vi "change CLFN properties.vi"() -> ()   [LabVIEW 2019]
uses:
  <vilib>/Utility/traverseref.llb/TRef TravTarget.ctl
  ca4436d5-b66f-4770-9057-43c195b94ee2.vi
  <vilib>/Utility/traverseref.llb/VI Scripting - Traverse.lvlib
panel:
  in  "Item(s) to Update":i32[](listbox)
  in  "PGconn/PGresults Type":enum16{"U32", "U64", "Pointer-Size"}(ring)
  out "Functions used":string[](array[string])
  in  "ShowMod":bool=TRUE caption="Open modified diagrams"
  in  "ApplyMod":bool=TRUE caption="Apply modifications"
  in  "Dynamic  Library":bool=TRUE
  in  "Call convention":enum16{"C", "stdcall"}(ring)
  in  "LibPath":string="libpq.*"
  out "Mod":path[](array[path]) caption="Modified VIs"
  in  "AnyThread":bool
  in  "folder":path=path "C:/dev/pq-labview"
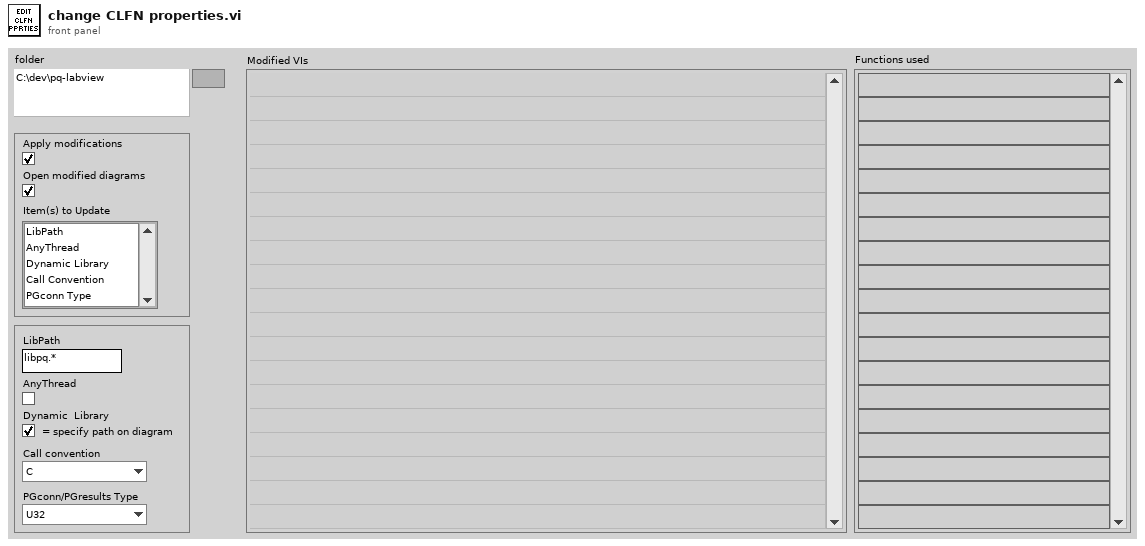
[diagram p1: front panel]
types:
  T1 = cluster{"AnyThread":bool, "LibPath":path, "Call Convention":u32, "Dynamic Library":bool, "PGconn Type":enum16{"I8", "I16", "I32", "I64", "U8", "U16", "U32", "U64", "SGL", "DBL", "PTR INT", "PTR UINT"}}
  T2 = enum16{"I8", "I16", "I32", "I64", "U8", "U16", "U32", "U64", "SGL", "DBL", "PTR INT", "PTR UINT"}
  T3 = typedef "TRef TravTarget.ctl" = enum16{"FP", "BD", "Other"}
  T4 = cluster{"Parameter Name":string, "Num Dimensions":i32, "Parameter Type":enum16{"Numeric", "Array", "String", "Waveform", "Digital Waveform", "Digital Table", "ActiveX", "Any", "Instance Data Pointer", "Void"}, "Numeric Type":enum16{"I8", "I16", "I32", "I64", "U8", "U16", "U32", "U64", "SGL", "DBL", "PTR INT", "PTR UINT"}, "Param Passing":enum16{"By Value", "Pointer To Value"}, "Array Passing":enum16{"Array Data Pointer", "Array Handle", "Array Handle Pointer"}, "String Passing":enum16{"C String Pointer", "Pascal String Pointer", "String Handle", "String Handle Pointer"}, "Adapt Format":enum16{"By Value", "Pointer To Value"}, "ActiveX Types":enum16{"ActiveX Variant Pointer", "IDispatch* Pointer", "IUnknown* Pointer"}, "Const (unused)":bool, "Minimum Size":string}[]
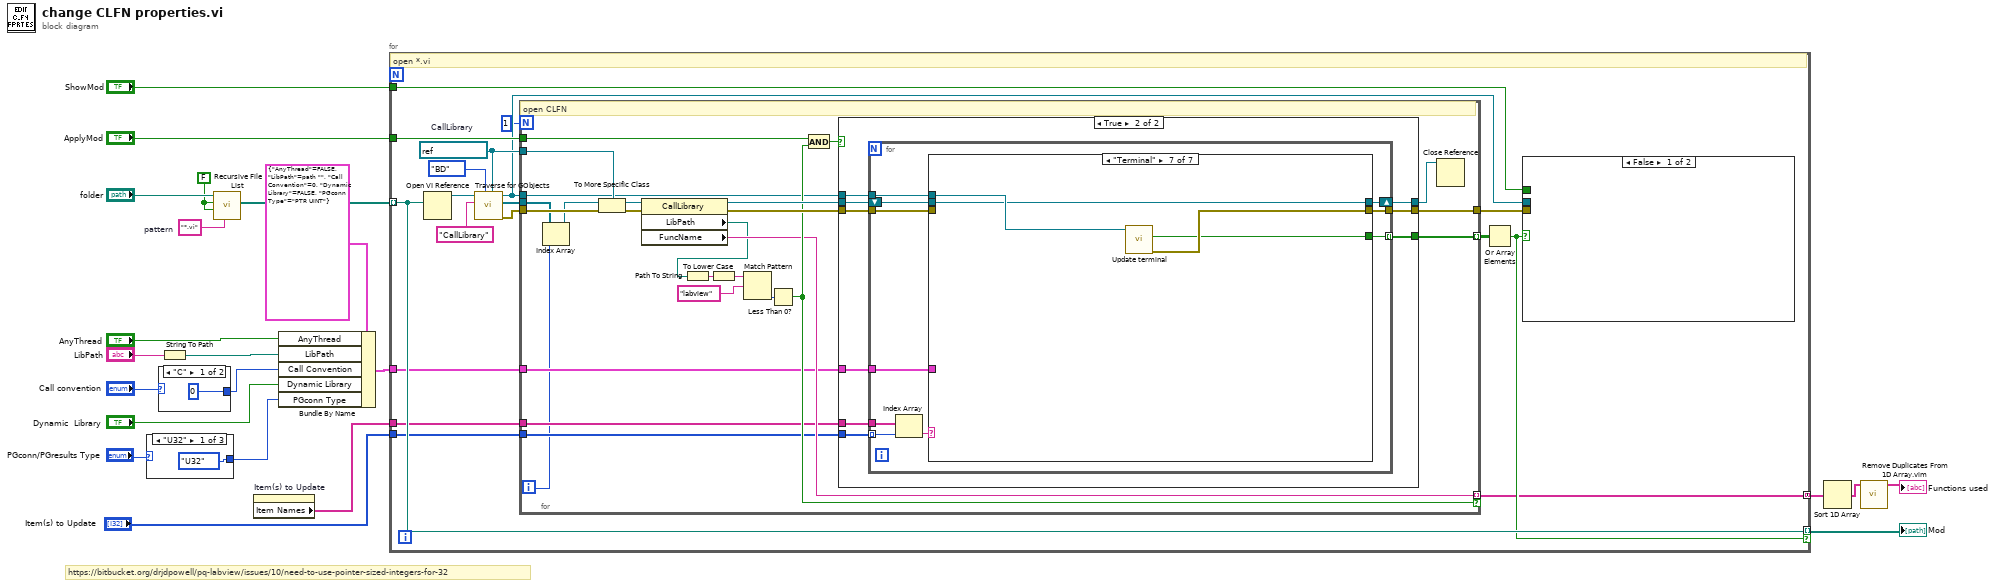
[diagram p0: block diagram]
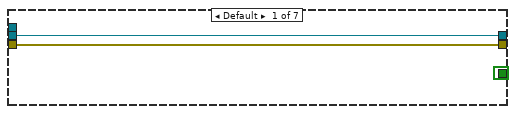
[diagram p3: hidden frame]
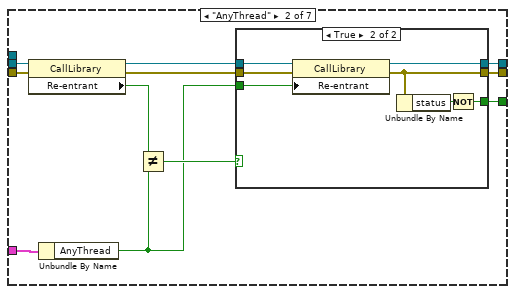
[diagram p4: hidden frame]
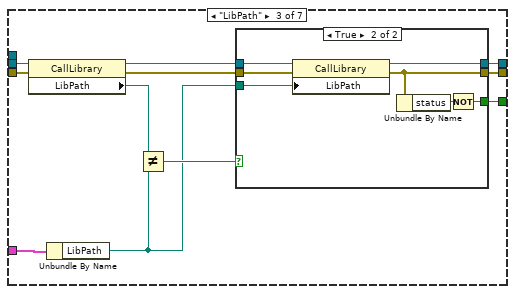
[diagram p6: hidden frame]
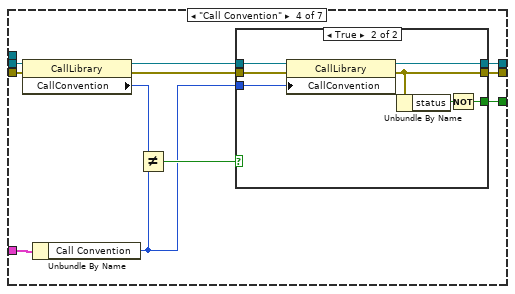
[diagram p8: hidden frame]
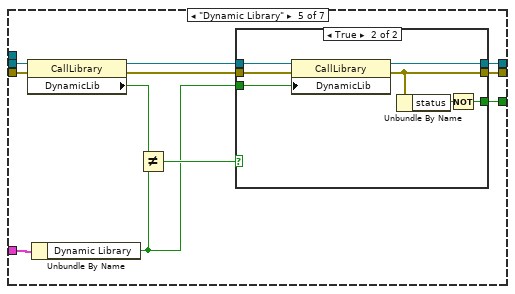
[diagram p10: hidden frame]
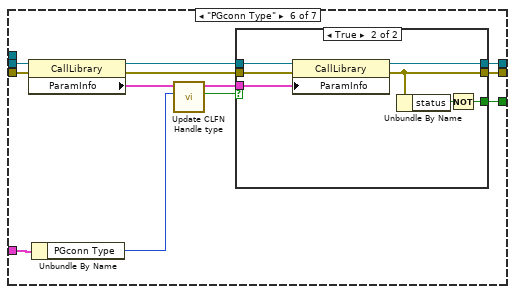
[diagram p12: hidden frame]
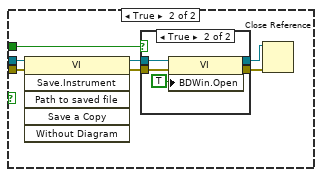
[diagram p14: hidden frame]
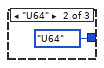
[diagram p16: hidden frame]
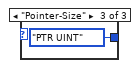
[diagram p17: hidden frame]
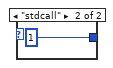
[diagram p18: hidden frame]
diagram:
  w20 = FALSE
  w19 = "*.vi"  # pattern
  # "https://bitbucket.org/drjdpowell/pq-labview/issues/10/need-to-use-pointer-sized-integers-for-32"
  n1 = case shown="\"U32\"" "PGconn/PGresults Type" {
    tunnel: [T2."U32" ("Numeric Type") T2."U64" ("Numeric Type") T2."PTR UINT" ("Numeric Type")] -> w4
    frame "U32" {
    }
    frame "U64" {
    }
    frame "Pointer-Size" {
    }
  }
  n2 = case shown="\"C\"" "Call convention" {
    tunnel: [u32 0 ("Calling Convention") u32 1 ("Calling Convention")] -> w6
    frame "C" {
    }
    frame "stdcall" {
    }
  }
  n3 = String To Path(string="LibPath") -> (path=w7:path)
  n4 = call <vilib>:"Recursive File List.vi"("pattern"=w19, "Continue Recursing on Error? (F)"=w20, "Treat LLBs as Folders?"=w20, "Folder Path"="folder") -> ("All Files in Dir"=w18:path[])  [unwired: 3 in, 4 out]
  n5 = property on="Item(s) to Update" class="LstBox (strict)"() -> ("Item Names"=w1:string[])  [unwired: 2 in, 2 out]
  n6 = Bundle By Name(cluster=T1 {"AnyThread"=FALSE, "LibPath"=path "", "Call Convention"=0, "Dynamic Library"=FALSE, "PGconn Type"=enum."PTR UINT"} ("output cluster"), "AnyThread"="AnyThread", "LibPath"=w7, "Call Convention"=w6, "Dynamic Library"="Dynamic  Library", "PGconn Type"=w4) -> (w5:T1)
  n7 = for {
    tunnel: w18 -> [w38] mode=indexing
    tunnel: [w38] -> w22 mode=indexing if=w34
    tunnel: "ApplyMod" -> [w37]
    tunnel: "ShowMod" -> [w36]
    tunnel: [w33] -> w13 mode=concatenating
    tunnel: w5 -> [w32]
    tunnel: "Item(s) to Update" -> [w31]
    tunnel: w1 -> [w30]
    w42 = refnum<vi> refnum  # CallLibrary
    # "open *.vi"
    n8 = Open VI Reference(vi path=w38) -> (vi reference=w45:refnum<vi>)  [unwired: 5 in, 1 out]
    n9 = call <vilib>:"Traverse for GObjects.vi"("Other Refnum"=w42, "Traverse Target"=TRef_TravTarget."BD", "Class Name"="CallLibrary", "VI Refnum"=w45) -> ("error out"=w41:errorcluster, "References"=w39:refnum<vi>[], "dup VI Refnum"=w29:refnum<vi>)  [unwired: 4 in, 1 out]
    n10 = for {
      N: 1 -> [_]
      tunnel: w39 -> [w46]
      tunnel: w42 -> [w70]
      tunnel: w41 -> [w69]
      tunnel: [w68] -> w40
      tunnel: w37 -> [w66]
      tunnel: [w65] -> w35 mode=indexing
      tunnel: [w54] -> w33 mode=indexing if=w55
      tunnel: w32 -> [w52]
      tunnel: w31 -> [w51]
      tunnel: w30 -> [w50]
      tunnel: w29 -> [w49]
      i -> [w48]
      # "open CLFN"
      n11 = Index Array(array=w46, index=w48) -> (element=w47:refnum<vi>)
      n12 = To More Specific Class(target class=w70, reference=w47, error in=w69) -> (specific class reference=w64:refnum<vi>, error out=w63:errorcluster)
      n13 = property class="CallLibrary"(reference=w64, error in=w63) -> (reference out=w62:refnum<vi>, error out=w61:errorcluster, "LibPath"=w53:path, "FuncName"=w54:string)
      n14 = Path To String(path=w53) -> (string=w60:string)
      n15 = To Lower Case(string=w60) -> (all lower case string=w59:string)
      n16 = Match Pattern(string=w59, regular expression="labview") -> (offset past match=w57:i32)  [unwired: 1 in, 3 out]
      n17 = Less Than 0?(x=w57) -> (x < 0?=w55:bool)
      n18 = Compound Arithmetic op=AND(w66, w55) -> (w56:bool)
      n19 = case shown="True" w56 {
        tunnel: w62 -> [w72 w79]
        tunnel: w61 -> [w71 w78]
        tunnel: [w71 w81] -> w68
        tunnel: [w72 w80] -> w67
        tunnel: [_ w77] -> w65
        tunnel: w52 -> [_ w76]
        tunnel: w51 -> [_ w75]
        tunnel: w50 -> [_ w74]
        tunnel: w49 -> [_ w73]
        frame False {
        }
        frame True {
          n20 = for {
            shift-right: [w90] -> w80
            shift-left: w79 -> [w89]
            tunnel: w78 -> [w88]
            tunnel: [w91] -> w81
            tunnel: [w87] -> w77 mode=indexing
            tunnel: w76 -> [w83]
            tunnel: w75 -> [w85] mode=indexing
            tunnel: w74 -> [w86]
            tunnel: w73 -> [w82]
            n21 = Index Array(array=w86, index=w85) -> (element=w84:string)
            n22 = case shown="\"Terminal\"" w84 {
              tunnel: [w93 w105 w125 w145 w165 w186 w198] -> w91
              tunnel: [w94 w104 w124 w144 w164 w185 w197] -> w90
              tunnel: w89 -> [w94 w103 w123 w143 w163 w184 w197]
              tunnel: w88 -> [w93 w100 w120 w140 w160 w181 _]
              tunnel: [FALSE w99 w119 w139 w159 w180 w196] -> w87
              tunnel: w83 -> [_ w98 w117 w137 w157 w177 _]
              tunnel: w82 -> [_ _ _ _ _ _ w199]
              frame Default {
              }
              frame "AnyThread" {
                n23 = property class="CallLibrary"(reference=w103, error in=w100) -> (reference out=w102:refnum<vi>, error out=w101:errorcluster, "Re-entrant"=w97:bool)
                n24 = Unbundle By Name(w98) -> ("AnyThread"=w95:bool)
                n25 = Not Equal?(x=w97, y=w95) -> (x != y?=w96:bool)
                n26 = case shown="True" w96 {
                  tunnel: [w106 w111] -> w105
                  tunnel: [w107 w114] -> w104
                  tunnel: w102 -> [w107 w113]
                  tunnel: w101 -> [w106 w112]
                  tunnel: [_ w109] -> w99
                  tunnel: w95 -> [_ w108]
                  frame False {
                  }
                  frame True {
                    n27 = property class="CallLibrary"(reference=w113, error in=w112, "Re-entrant"=w108) -> (reference out=w114:refnum<vi>, error out=w111:errorcluster)
                    n28 = Unbundle By Name(w111) -> ("status"=w110:bool)
                    n29 = Not(x=w110) -> (.not. x?=w109:bool)
                  }
                }
              }
              frame "LibPath" {
                n30 = property class="CallLibrary"(reference=w123, error in=w120) -> (reference out=w122:refnum<vi>, error out=w121:errorcluster, "LibPath"=w116:path)
                n31 = Unbundle By Name(w117) -> ("LibPath"=w115:path)
                n32 = Not Equal?(x=w116, y=w115) -> (x != y?=w118:bool)
                n33 = case shown="True" w118 {
                  tunnel: [w126 w131] -> w125
                  tunnel: [w127 w134] -> w124
                  tunnel: w122 -> [w127 w133]
                  tunnel: w121 -> [w126 w132]
                  tunnel: [_ w129] -> w119
                  tunnel: w115 -> [_ w128]
                  frame False {
                  }
                  frame True {
                    n34 = property class="CallLibrary"(reference=w133, error in=w132, "LibPath"=w128) -> (reference out=w134:refnum<vi>, error out=w131:errorcluster)
                    n35 = Unbundle By Name(w131) -> ("status"=w130:bool)
                    n36 = Not(x=w130) -> (.not. x?=w129:bool)
                  }
                }
              }
              frame "Call Convention" {
                n37 = property class="CallLibrary"(reference=w143, error in=w140) -> (reference out=w142:refnum<vi>, error out=w141:errorcluster, "CallConvention"=w136:u32)
                n38 = Unbundle By Name(w137) -> ("Call Convention"=w135:u32)
                n39 = Not Equal?(x=w136, y=w135) -> (x != y?=w138:bool)
                n40 = case shown="True" w138 {
                  tunnel: [w146 w151] -> w145
                  tunnel: [w147 w154] -> w144
                  tunnel: w142 -> [w147 w153]
                  tunnel: w141 -> [w146 w152]
                  tunnel: [_ w149] -> w139
                  tunnel: w135 -> [_ w148]
                  frame False {
                  }
                  frame True {
                    n41 = property class="CallLibrary"(reference=w153, error in=w152, "CallConvention"=w148) -> (reference out=w154:refnum<vi>, error out=w151:errorcluster)
                    n42 = Unbundle By Name(w151) -> ("status"=w150:bool)
                    n43 = Not(x=w150) -> (.not. x?=w149:bool)
                  }
                }
              }
              frame "Dynamic Library" {
                n44 = property class="CallLibrary"(reference=w163, error in=w160) -> (reference out=w162:refnum<vi>, error out=w161:errorcluster, "DynamicLib"=w156:bool)
                n45 = Unbundle By Name(w157) -> ("Dynamic Library"=w155:bool)
                n46 = Not Equal?(x=w156, y=w155) -> (x != y?=w158:bool)
                n47 = case shown="True" w158 {
                  tunnel: [w166 w171] -> w165
                  tunnel: [w167 w174] -> w164
                  tunnel: w162 -> [w167 w173]
                  tunnel: w161 -> [w166 w172]
                  tunnel: [_ w169] -> w159
                  tunnel: w155 -> [_ w168]
                  frame False {
                  }
                  frame True {
                    n48 = property class="CallLibrary"(reference=w173, error in=w172, "DynamicLib"=w168) -> (reference out=w174:refnum<vi>, error out=w171:errorcluster)
                    n49 = Unbundle By Name(w171) -> ("status"=w170:bool)
                    n50 = Not(x=w170) -> (.not. x?=w169:bool)
                  }
                }
              }
              frame "PGconn Type" {
                n51 = property class="CallLibrary"(reference=w184, error in=w181) -> (reference out=w183:refnum<vi>, error out=w182:errorcluster, "ParamInfo"=w178:T4)
                n52 = Unbundle By Name(w177) -> ("PGconn Type"=w176:T2)
                n53 = call "Update CLFN Handle type.vi"("Numeric Type"=w176, "ParamInfo"=w178) -> ("Change"=w175:bool, "ParamInfo"=w179:T4)  [unwired: 8 in]
                n54 = case shown="True" w175 {
                  tunnel: [w187 w192] -> w186
                  tunnel: [w188 w195] -> w185
                  tunnel: w183 -> [w188 w194]
                  tunnel: w182 -> [w187 w193]
                  tunnel: [_ w190] -> w180
                  tunnel: w179 -> [_ w189]
                  frame False {
                  }
                  frame True {
                    n55 = property class="CallLibrary"(reference=w194, error in=w193, "ParamInfo"=w189) -> (reference out=w195:refnum<vi>, error out=w192:errorcluster)
                    n56 = Unbundle By Name(w192) -> ("status"=w191:bool)
                    n57 = Not(x=w191) -> (.not. x?=w190:bool)
                  }
                }
              }
              frame "Terminal" {
                n58 = call "Update terminal.vi"("VI in"=w199) -> ("error out"=w198:errorcluster, "change?"=w196:bool)  [unwired: 9 in]
              }
            }
          }
        }
      }
      n59 = Close Reference(reference=w67) -> ()  [unwired: 1 in, 1 out]
    }
    n60 = Or Array Elements(Boolean array=w35) -> (logical OR=w34:bool)
    n61 = case shown="False" w34 {
      tunnel: w40 -> [_ w206]
      tunnel: w29 -> [_ w205]
      tunnel: w36 -> [_ w200]
      frame False {
      }
      frame True {
        n62 = invoke class="VI" method="Save.Instrument"(reference=w205, error in=w206) -> (reference out=w203:refnum<vi>, error out=w204:errorcluster)  [unwired: 4 in, 4 out]
        n63 = case shown="True" w200 {
          tunnel: w204 -> [w207 w213]
          tunnel: w203 -> [w208 w212]
          tunnel: [w208 w211] -> w202
          tunnel: [w207 w210] -> w201
          frame False {
          }
          frame True {
            n64 = property class="VI"(reference=w212, error in=w213, "BDWin.Open"=TRUE ("Block Diagram Window:Open")) -> (reference out=w211:refnum<vi>, error out=w210:errorcluster)
          }
        }
        n65 = Close Reference(reference=w202, error in (no error)=w201) -> ()  [unwired: 1 out]
      }
    }
  }
  "Mod" <- w22
  n66 = Sort 1D Array(array=w13) -> (sorted array=w12:string[])
  n67 = call "Remove Duplicates From 1D Array.vim"("array"=w12) -> ("array with duplicates removed"=→"Functions used":string[])  [unwired: 10 in]
